vi "Generate Archive Locations.vi"(9 "Archive?":bool, 10 "Key":string, 11 "Archivist In":refnum<class "Archivist.lvclass">) -> (2 "Path Out":path, 3 "Archivist Out":refnum<class "Archivist.lvclass">)   [LabVIEW 2019, in "Archivist.lvclass"]
uses:
  Archivist.lvclass
  Archivist.lvclass/Archivist.ctl
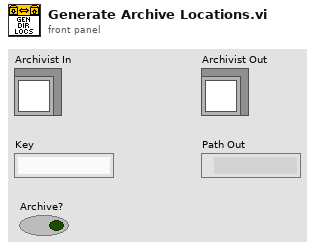
[diagram p1: front panel]
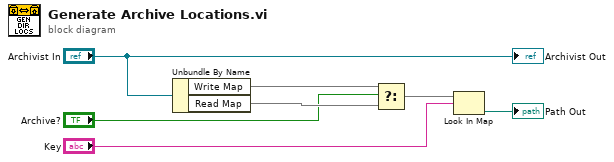
[diagram p0: block diagram]
diagram:
  n1 = Unbundle By Name("Archivist In") -> ("Write Map"=w6:map{string, path}, "Read Map"=w5:map{string, path})
  n2 = Select(t=w6, s="Archive?", f=w5) -> (s? t:f=w3:map{string, path})
  n3 = Look In Map(map=w3, key="Key") -> (value=→"Path Out":path)  [unwired: 1 in, 1 out]
  "Archivist Out" <- "Archivist In"
